vi "measure OBW Measurement.vi"(8 "error in (no error)":errorcluster, 11 "SA Measurement in":refnum<class "SA Measurement.lvclass">) -> (0 "error out":errorcluster, 3 "SA Measurement out":refnum<class "SA Measurement.lvclass">)   [LabVIEW 2023, in "Spectrum Analyzer.lvlib" / "SA Measurement.lvclass"]
uses:
  SA Measurement.lvclass
  SA Measurement.lvclass/SA Measurement.ctl
  TYPE DEFINITION/Keysight 9020A/TYPE Measurement Preset.ctl
  Spectrum Analyzer.lvlib
  TYPE DEFINITION/TYPE RBW and VBW Select.ctl
  Interface_Spectrum/Interface_Spectrum.lvclass
  TYPE DEFINITION/TYPE Marker Peak Search Type.ctl
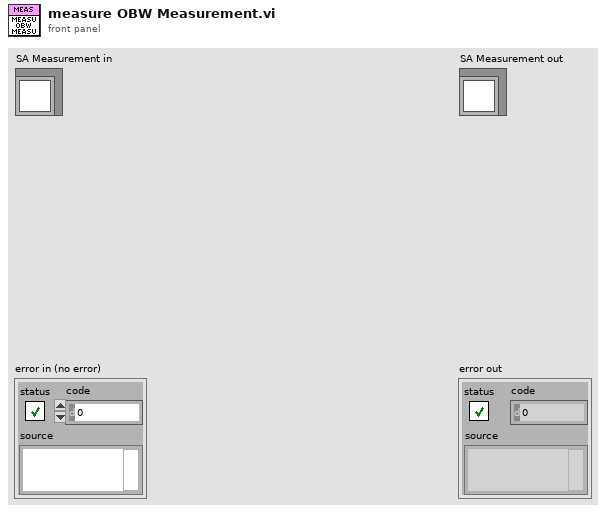
[diagram p1: front panel]
types:
  T1 = typedef "Spectrum Analyzer.lvlib/TYPE Marker Peak Search Type.ctl" = enum16{"Max", "Next Peak"}
  T2 = typedef "Spectrum Analyzer.lvlib/TYPE RBW and VBW Select.ctl" = enum16{"Res BW", "Video BW"}
  T3 = typedef "Spectrum Analyzer.lvlib/TYPE Measurement Preset.ctl" = enum16{"Sweep SA Mode", "Channel Power", "Occupied BW", "ACP", "Spurious Emission", "Spurious Emission Mask", "Burst Power (Transmit Power)"}
  T4 = typedef "Spectrum Analyzer.lvlib/TYPE Y-axis Unit.ctl" = enum16{"dBm", "dBmV", "dBuV", "dBpW", "Volt", "Ampere", "Watt"}
  T5 = typedef "Spectrum Analyzer.lvlib/TYPE Reference Level and Atten Param.ctl" = cluster{"Reference Level":dbl, "Atten":i32, "Atten Auto?":bool, "Reference Level Offset":dbl}
  T6 = typedef "Spectrum Analyzer.lvlib/TYPE Display Trace Mode Select.ctl" = enum16{"Clear Write", "Max Hold", "Min Hold", "Average", "View"}
  T7 = typedef "Spectrum Analyzer.lvlib/TYPE Detect Mode Select.ctl" = enum16{"Det Auto (Normal)", "Auto Peak", "Positive Peak", "Negative Peak", "Sample", "RMS", "Average", "Quasipeak", "CISPR Average", "RMS Average"}
  T8 = cluster{"Trace Mode":T6, "Detector Type":T7, "Detect Auto?":bool}[]
  T9 = typedef "Spectrum Analyzer.lvlib/TYPE Marker Value.ctl" = cluster{"X-axis":dbl, "Y-axis":dbl}
  T10 = typedef "Spectrum Analyzer.lvlib/TYPE OBW Measurement.ctl" = cluster{"Occupied BW (Hz)":dbl, "Total Power or OBW Power - dBm":dbl, "Transmit Frequency Error (Hz)":dbl, "x DB Bandwidth (Hz)":dbl, "Lower OBW Frequency (Hz)":dbl, "Upper OBW Frequency (Hz)":dbl}
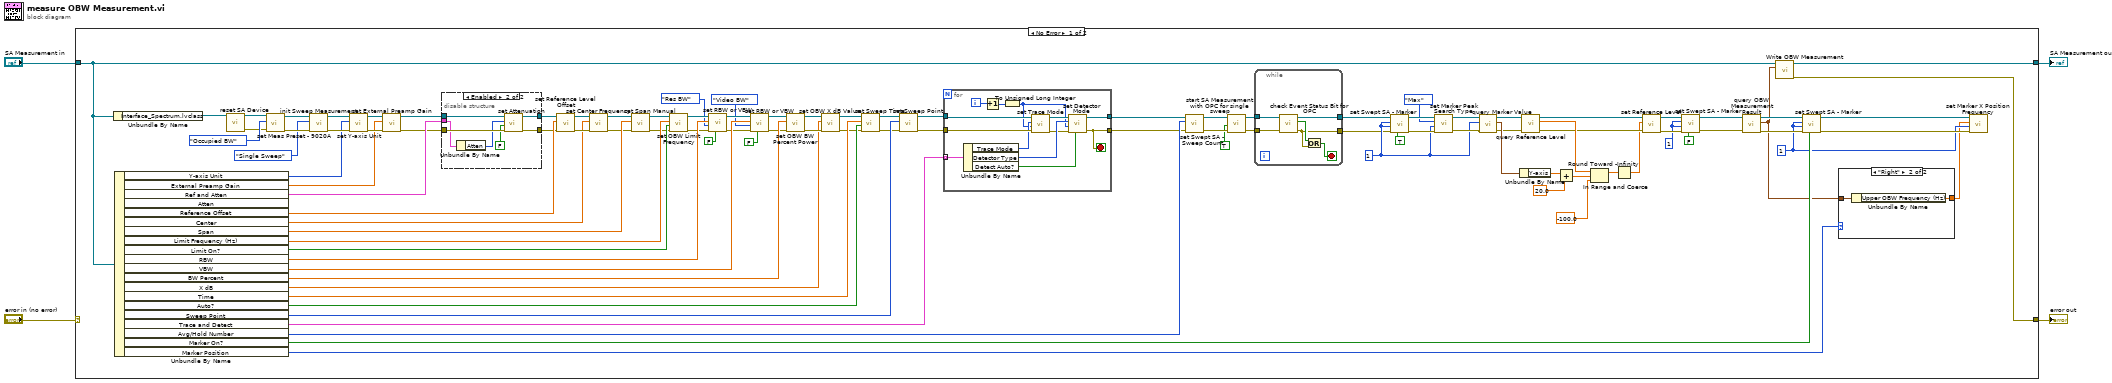
[diagram p0: block diagram]
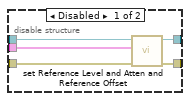
[diagram p2: hidden frame]
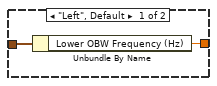
[diagram p3: hidden frame]
diagram:
  n1 = case shown="No Error" "error in (no error)" {
    selector: "error in (no error)" -> [_ w143]
    tunnel: [w45 w143] -> w3
    tunnel: [w46 w142] -> w1
    tunnel: "SA Measurement in" -> [w47 w142]
    frame No Error {
      w9 = 1 ("Index")
      w25 = 1 ("Index")
      w37 = 1 ("Index")
      n2 = Unbundle By Name(w47) -> ("Interface_Spectrum.lvclass"=w87:refnum<class "Interface_Spectrum.lvclass">)
      n3 = Unbundle By Name(w47) -> ("Y-axis Unit"=w95:T4, "External Preamp Gain"=w80:dbl, "Ref and Atten"=w102:T5, "Reference Offset"=w101:dbl, "Center"=w98:dbl, "Span"=w72:dbl, "Limit Frequency (Hz)"=w79:dbl, "Limit On?"=w78:bool, "RBW"=w67:dbl, "VBW"=w61:dbl, "BW Percent"=w77:dbl, "X dB"=w74:dbl, "Time"=w55:dbl, "Auto?"=w54:bool, "Sweep Point"=w50:u32, "Trace and Detect"=w94:T8, "Avg/Hold Number"=w93:u32, "Marker On?"=w42:bool, "Marker Position"=w41:enum16{"Left", "Right"})  [unwired: 1 out]
      n4 = call-dynamic "reset SA Device.vi"("Interface_Spectrum in"=w87) -> ("error out"=w85:errorcluster, "Interface_Spectrum out"=w86:refnum<class "Interface_Spectrum.lvclass">)  [unwired: 9 in]
      n5 = call-dynamic "set Meas Preset - 9020A.vi"("error in (no error)"=w85, "Measurement Preset"=TYPE_Measurement_Preset."Occupied BW", "Interface_Spectrum in"=w86) -> ("error out"=w104:errorcluster, "Interface_Spectrum out"=w105:refnum<class "Interface_Spectrum.lvclass">)  [unwired: 7 in]
      n6 = call-dynamic "init Sweep Measurement.vi"("error in (no error)"=w104, "Sweep Measurement Mode"=enum16{"Single Sweep", "Continuous Sweep"}."Single Sweep", "Interface_Spectrum in"=w105) -> ("error out"=w96:errorcluster, "Interface_Spectrum out"=w97:refnum<class "Interface_Spectrum.lvclass">)  [unwired: 7 in]
      n7 = call-dynamic "set Y-axis Unit.vi"("error in (no error)"=w96, "Y-axis Unit"=w95, "Interface_Spectrum in"=w97) -> ("error out"=w83:errorcluster, "Interface_Spectrum out"=w84:refnum<class "Interface_Spectrum.lvclass">)  [unwired: 7 in]
      n8 = call-dynamic "set External Preamp Gain.vi"("error in (no error)"=w83, "External Preamp Gain (dB)"=w80, "Interface_Spectrum in"=w84) -> ("error out"=w81:errorcluster, "Interface_Spectrum out"=w82:refnum<class "Interface_Spectrum.lvclass">)  [unwired: 7 in]
      n9 = disable-structure shown="Enabled" {
        disable-tunnel: w102 -> [w111 w114]
        disable-tunnel: w82 -> [w110 w118]
        disable-tunnel: w81 -> [w109 w117]
        disable-tunnel: [w108 w116] -> w35
        disable-tunnel: [w107 w115] -> w34
        frame Disabled {
          n10 = call-dynamic "set Reference Level and Atten and Reference Offset.vi"("error in (no error)"=w109, "Reference Level, Atten, Reference Offset"=w111, "Interface_Spectrum in"=w110) -> ("error out"=w107:errorcluster, "Interface_Spectrum out"=w108:refnum<class "Interface_Spectrum.lvclass">)  [unwired: 7 in]
        }
        frame Enabled {
          n11 = Unbundle By Name(w114) -> ("Atten"=w113:i32)
          n12 = call-dynamic "set Attenuation.vi"("error in (no error)"=w117, "Auto?"=FALSE, "Attenuation"=w113, "Interface_Spectrum in"=w118) -> ("error out"=w115:errorcluster, "Interface_Spectrum out"=w116:refnum<class "Interface_Spectrum.lvclass">)  [unwired: 6 in]
        }
      }
      n13 = call-dynamic "set Reference Level Offset.vi"("error in (no error)"=w34, "Reference Level Offset"=w101, "Interface_Spectrum in"=w35) -> ("error out"=w99:errorcluster, "Interface_Spectrum out"=w100:refnum<class "Interface_Spectrum.lvclass">)  [unwired: 7 in]
      n14 = call-dynamic "set Center Frequency.vi"("error in (no error)"=w99, "Center Frequency (Hz)"=w98, "Interface_Spectrum in"=w100) -> ("error out"=w71:errorcluster, "Interface_Spectrum out"=w73:refnum<class "Interface_Spectrum.lvclass">)  [unwired: 7 in]
      n15 = call-dynamic "set Span Manual.vi"("error in (no error)"=w71, "Span (Hz)"=w72, "Interface_Spectrum in"=w73) -> ("error out"=w69:errorcluster, "Interface_Spectrum out"=w70:refnum<class "Interface_Spectrum.lvclass">)  [unwired: 7 in]
      n16 = call-dynamic "set OBW Limit Frequency.vi"("error in (no error)"=w69, "Limit On?"=w78, "Limit Frequency (Hz)"=w79, "Interface_Spectrum in"=w70) -> ("error out"=w65:errorcluster, "Interface_Spectrum out"=w68:refnum<class "Interface_Spectrum.lvclass">)  [unwired: 6 in]
      n17 = call-dynamic "set RBW or VBW.vi"("BW Auto?"=FALSE, "error in (no error)"=w65, "BW Type"=TYPE_RBW_and_VBW_Select."Res BW", "BW Value (Hz)"=w67, "Interface_Spectrum in"=w68) -> ("error out"=w59:errorcluster, "Interface_Spectrum out"=w62:refnum<class "Interface_Spectrum.lvclass">)  [unwired: 5 in]
      n18 = call-dynamic "set RBW or VBW.vi"("BW Auto?"=FALSE, "error in (no error)"=w59, "BW Type"=TYPE_RBW_and_VBW_Select."Video BW", "BW Value (Hz)"=w61, "Interface_Spectrum in"=w62) -> ("error out"=w57:errorcluster, "Interface_Spectrum out"=w58:refnum<class "Interface_Spectrum.lvclass">)  [unwired: 5 in]
      n19 = call-dynamic "set OBW BW Percent Power.vi"("error in (no error)"=w57, "OBW BW % Pwr"=w77, "Interface_Spectrum in"=w58) -> ("error out"=w75:errorcluster, "Interface_Spectrum out"=w76:refnum<class "Interface_Spectrum.lvclass">)  [unwired: 7 in]
      n20 = call-dynamic "set OBW X dB Value.vi"("error in (no error)"=w75, "OBW X dB (minus Value)"=w74, "Interface_Spectrum in"=w76) -> ("error out"=w53:errorcluster, "Interface_Spectrum out"=w56:refnum<class "Interface_Spectrum.lvclass">)  [unwired: 7 in]
      n21 = call-dynamic "set Sweep Time.vi"("error in (no error)"=w53, "Sweep Time Auto?"=w54, "Sweep Time(sec)"=w55, "Interface_Spectrum in"=w56) -> ("error out"=w49:errorcluster, "Interface_Spectrum out"=w52:refnum<class "Interface_Spectrum.lvclass">)  [unwired: 6 in]
      n22 = call-dynamic "set Sweep Point.vi"("error in (no error)"=w49, "Sweep Point"=w50, "Interface_Spectrum in"=w52) -> ("error out"=w48:errorcluster, "Interface_Spectrum out"=w51:refnum<class "Interface_Spectrum.lvclass">)  [unwired: 7 in]
      n23 = for {
        tunnel: w51 -> [w140]
        tunnel: w48 -> [w139]
        tunnel: w94 -> [w141] mode=indexing
        tunnel: [w129] -> w32
        tunnel: [w130] -> w33
        i -> [w138]
        stop <- w129 stop-if-true
        n24 = Unbundle By Name(w141) -> ("Trace Mode"=w136:T6, "Detector Type"=w134:T7, "Detect Auto?"=w131:bool)
        n25 = Increment(x=w138) -> (x+1=w137:i32)
        n26 = To Unsigned Long Integer(number=w137) -> (unsigned 32bit integer=w132:u32)
        n27 = call-dynamic "set Trace Mode.vi"("error in (no error)"=w139, "Trace Index"=w132, "Trace Mode"=w136, "Interface_Spectrum in"=w140) -> ("error out"=w133:errorcluster, "Interface_Spectrum out"=w135:refnum<class "Interface_Spectrum.lvclass">)  [unwired: 6 in]
        n28 = call-dynamic "set Detector Mode.vi"("Detect Auto?"=w131, "error in (no error)"=w133, "Trace Index"=w132, "Detector Type"=w134, "Interface_Spectrum in"=w135) -> ("error out"=w129:errorcluster, "Interface_Spectrum out"=w130:refnum<class "Interface_Spectrum.lvclass">)  [unwired: 5 in]
      }
      n29 = call-dynamic "set Swept SA - Sweep Count.vi"("error in (no error)"=w32, "Sweep Count"=w93, "Interface_Spectrum in"=w33) -> ("error out"=w91:errorcluster, "Interface_Spectrum out"=w92:refnum<class "Interface_Spectrum.lvclass">)  [unwired: 7 in]
      n30 = call-dynamic "start SA Measurement with OPC for single sweep.vi"("error in (no error)"=w91, "with OPC?"=TRUE, "Interface_Spectrum in"=w92) -> ("error out"=w88:errorcluster, "Interface_Spectrum out"=w89:refnum<class "Interface_Spectrum.lvclass">)  [unwired: 7 in]
      n31 = while {
        tunnel: w89 -> [w128]
        tunnel: w88 -> [w127]
        tunnel: [w124] -> w7
        tunnel: [w123] -> w8
        stop <- w125 stop-if-true
        n32 = call-dynamic "check Event Status Bit for OPC.vi"("error in (no error)"=w127, "Interface_Spectrum in"=w128) -> ("error out"=w124:errorcluster, "OPC Bit Changed?"=w126:bool, "Interface_Spectrum out"=w123:refnum<class "Interface_Spectrum.lvclass">)  [unwired: 7 in]
        n33 = Or(x=w126, y=w124) -> (x .or. y?=w125:bool)
      }
      n34 = call-dynamic "set Swept SA - Marker.vi"("On?"=TRUE, "error in (no error)"=w7, "trace"=w25, "Index"=w25, "Interface_Spectrum in"=w8) -> ("error out"=w29:errorcluster, "Interface_Spectrum out"=w30:refnum<class "Interface_Spectrum.lvclass">)  [unwired: 5 in]
      n35 = call-dynamic "set Marker Peak Search Type.vi"("error in (no error)"=w29, "Marker Index"=w25, "Peak Search Type"=TYPE_Marker_Peak_Search_Type."Max", "Interface_Spectrum in"=w30) -> ("error out"=w26:errorcluster, "Interface_Spectrum out"=w27:refnum<class "Interface_Spectrum.lvclass">)  [unwired: 6 in]
      n36 = call-dynamic "query Marker Value.vi"("error in (no error)"=w26, "Marker Index"=w25, "Interface_Spectrum in"=w27) -> ("error out"=w20:errorcluster, "Marker Value"=w22:T9, "Interface_Spectrum out"=w21:refnum<class "Interface_Spectrum.lvclass">)  [unwired: 6 in]
      n37 = Unbundle By Name(w22) -> ("Y-axis"=w24:dbl)
      n38 = call-dynamic "query Reference Level.vi"("error in (no error)"=w20, "Interface_Spectrum in"=w21) -> ("error out"=w15:errorcluster, "Ref Level"=w18:dbl, "Interface_Spectrum out"=w19:refnum<class "Interface_Spectrum.lvclass">)  [unwired: 7 in]
      n39 = Add(x=w24, y=20.0) -> (x+y=w17:dbl)
      n40 = In Range and Coerce(upper limit=w18, x=w17, lower limit=-100.0) -> (coerced(x)=w14:dbl)  [unwired: 1 out]
      n41 = Round Toward -Infinity(1:w14) -> (0:w13:dbl)
      n42 = call-dynamic "set Reference Level.vi"("error in (no error)"=w15, "Reference Level"=w13, "Interface_Spectrum in"=w19) -> ("error out"=w11:errorcluster, "Interface_Spectrum out"=w12:refnum<class "Interface_Spectrum.lvclass">)  [unwired: 7 in]
      n43 = call-dynamic "set Swept SA - Marker.vi"("On?"=FALSE, "error in (no error)"=w11, "trace"=w9, "Index"=w9, "Interface_Spectrum in"=w12) -> ("error out"=w5:errorcluster, "Interface_Spectrum out"=w6:refnum<class "Interface_Spectrum.lvclass">)  [unwired: 5 in]
      n44 = call-dynamic "query OBW Measurement Result.vi"("error in (no error)"=w5, "Interface_Spectrum in"=w6) -> ("error out"=w43:errorcluster, "OBW Measurement"=w40:T10, "Interface_Spectrum out"=w44:refnum<class "Interface_Spectrum.lvclass">)  [unwired: 7 in]
      n45 = call "Write OBW Measurement.vi"("OBW Measurement"=w40, "SA Measurement in"=w47) -> ("error out"=w45:errorcluster, "SA Measurement out"=w46:refnum<class "SA Measurement.lvclass">)  [unwired: 8 in]
      n46 = call-dynamic "set Swept SA - Marker.vi"("On?"=w42, "error in (no error)"=w43, "trace"=w37, "Index"=w37, "Interface_Spectrum in"=w44) -> ("error out"=w38:errorcluster, "Interface_Spectrum out"=w39:refnum<class "Interface_Spectrum.lvclass">)  [unwired: 5 in]
      n47 = case shown="\"Right\"" w41 {
        tunnel: w40 -> [w120 w122]
        tunnel: [w119 w121] -> w36
        frame "Left", Default {
          n48 = Unbundle By Name(w120) -> ("Lower OBW Frequency (Hz)"=w119:dbl)
        }
        frame "Right" {
          n49 = Unbundle By Name(w122) -> ("Upper OBW Frequency (Hz)"=w121:dbl)
        }
      }
      n50 = call-dynamic "set Marker X Position Frequency.vi"("error in (no error)"=w38, "Index"=w37, "X Position Frequency (Hz)"=w36, "Interface_Spectrum in"=w39) -> ()  [unwired: 6 in, 2 out]
    }
    frame Error {
    }
  }
  "error out" <- w3
  "SA Measurement out" <- w1
